vi "Read PLC.vi"(8 "error in (no error)":errorcluster, 11 "Submodule EOL configuration in":refnum<class "Submodule EOL configuration.lvclass">) -> (0 "error out":errorcluster, 2 "PLC":T1={"PLC Folder Names"=[["Station0_Rx", "OP50A_TesterRxSignals"], ["Station0_Tx", "OP50A_TesterTxSignals"], ["Station1_Rx", "OP50B_TesterRxSignals"], ["Station1_Tx", "OP50B_TesterTxSignals"], ["Station2_Rx", "OP60A_TesterRxSignals"], ["Station2_Tx", "OP60A_TesterTxSignals"], ["Station3_Rx", "OP60B_TesterRxSignals"], ["Station3_Tx", "OP60B_TesterTxSignals"], ["Station4_Rx", "OP70A_TesterRxSignals"], ["Station4_Tx", "OP70A_TesterTxSignals"], ["Station5_Rx", "OP70B_TesterRxSignals"], ["Station5_Tx", "OP70B_TesterTxSignals"]], "PLC URL"="opc.tcp://localhost:49580 ", "Ignition Folder Names"=[["Ignition0_Rx", "[Submodule_EOL]/StaA/TesterRx"], ["Ignition0_Tx", "[Submodule_EOL]/StaA/TesterTx"], ["Ignition1_Rx", "[Submodule_EOL]/StaB/TesterRx"], ["Ignition1_Tx", "[Submodule_EOL]/StaB/TesterTx"], ["Ignition2_Rx", "[Submodule_EOL]/StaC/TesterRx"], ["Ignition2_Tx", "[Submodule_EOL]/StaC/TesterTx"], ["Ignition3_Rx", "[Submodule_EOL]/StaD/TesterRx"], ["Ignition3_Tx", "[Submodule_EOL]/StaD/TesterTx"], ["Ignition4_Rx", "[Submodule_EOL]/StaE/TesterRx"], ["Ignition4_Tx", "[Submodule_EOL]/StaE/TesterTx"], ["Ignition5_Rx", "[Submodule_EOL]/StaF/TesterRx"], ["Ignition5_Tx", "[Submodule_EOL]/StaF/TesterTx"]], "Ignition URL"="opc.tcp://10.64.0.22:62541/discovery", "Test Name"="Battery Submodule EOL"}, 3 "Submodule EOL configuration out":refnum<class "Submodule EOL configuration.lvclass">)   [LabVIEW 2025, in "Submodule EOL.lvlib" / "Submodule EOL configuration.lvclass"]
uses:
  Submodule EOL configuration.lvclass
  Submodule EOL configuration.lvclass/Submodule EOL configuration.ctl
  PLC.ctl
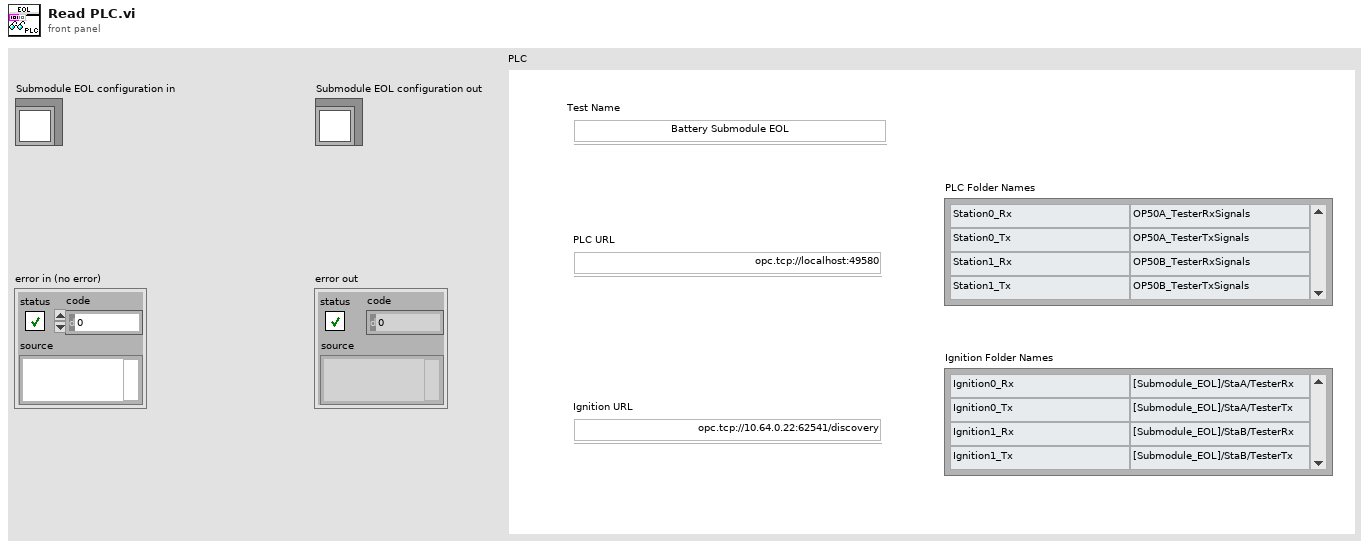
[diagram p1: front panel]
types:
  T1 = typedef "Submodule EOL.lvlib/Submodule EOL configuration.lvclass/PLC.ctl" = cluster{"PLC Folder Names":string[][], "PLC URL":string, "Ignition Folder Names":string[][], "Ignition URL":string, "Test Name":string}
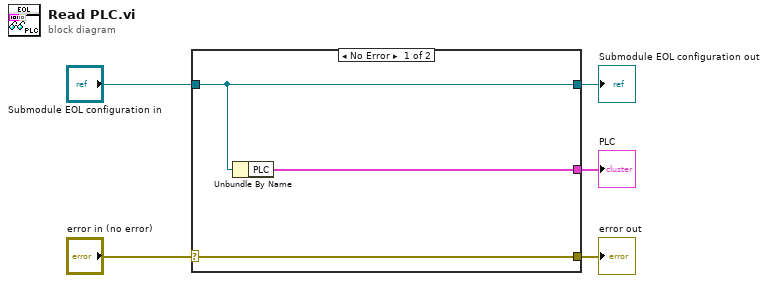
[diagram p0: block diagram]
diagram:
  n1 = case shown="No Error" "error in (no error)" {
    selector: "error in (no error)" -> [w8 w9]
    tunnel: [w8 w9] -> w4
    tunnel: [w7 w10] -> w2
    tunnel: "Submodule EOL configuration in" -> [w7 w10]
    tunnel: [w6 _] -> w1
    frame No Error {
      n2 = Unbundle By Name(w7) -> ("PLC"=w6:T1)
    }
    frame Error {
    }
  }
  "error out" <- w4
  "Submodule EOL configuration out" <- w2
  "PLC" <- w1
